vi "Main.vi"() -> ()   [LabVIEW 2020, in "DocTool.lvlib"]
uses:
  DocTool.lvlib
  TDefs/FP Items Properties Addendum.ctl
  TDefs/FP Items Properties.ctl
  TDefs/FP Item Properties.ctl
  TDefs/CopyTag.ctl
  TDefs/Single File Properties.ctl
  TDefs/Context.ctl
  Events/Events.ctl
  Events/UserEvent.ctl
  TDefs/State.ctl
  TDefs/States.ctl
  StateMachine.lvlib
panel:
  out "Status":string
  in  "Tab":enum32{"File Properties", "FP Items Properties"}(tab)
  out "Curr File":u16(slide) min=1 max=5 step=1 scale=1.0..5.0
  in  "Write FP":bool
  out "Total Files":u16
  in  "Copy_Desc":T1
  in  "Copy_HelpPath":T1
  in  "Copy_HelpTag":T1
  in  "File Properties":T2
  in  "PREV":bool
  in  "NEXT":bool
  in  "Read Folder":bool
  in  "Folder Path":path
  in  "SAVE":bool
  in  "Generate Help Tag":bool
  in  "Write":bool
  in  "Read File":bool
  out "FP VI Pic":picture
  out "BD VI Pic":picture
  in  "Connector Pane Terminals Only":bool
  in  "Tab Inputs":enum32{"Input", "More..."}(tab)
  in  "Inputs":T3
  in  "Input Addendum":T5
  in  "Tab Outputs":enum32{"Output", "More..."}(tab)
  in  "Outputs":T3
  in  "Output Addendum":T5
  in  "Mode":enum16{"All Items", "Selected Items"}(ring)
  in  "All":T1
  in  "Copy Descs to Tips":bool
  in  "Ignore Error Clusters":bool
  in  "Stop":bool
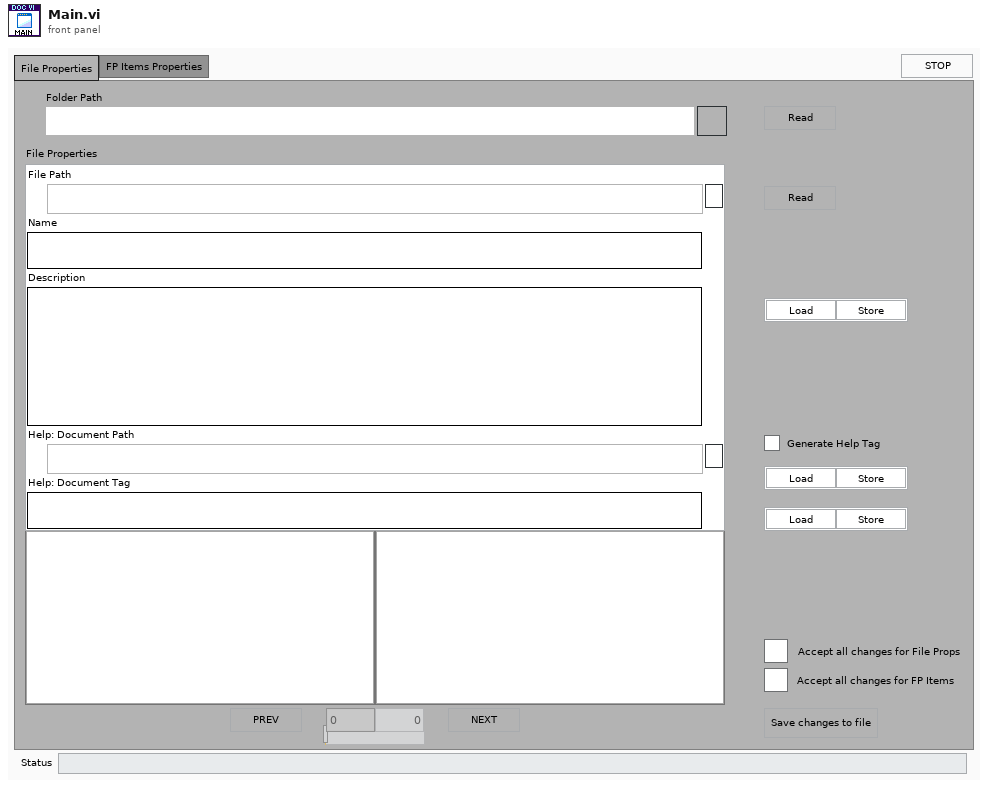
[diagram p1: front panel]
types:
  T1 = typedef "DocTool.lvlib/CopyTag.ctl" = cluster{"Load":bool, "Store":bool}
  T2 = typedef "DocTool.lvlib/Single File Properties.ctl" = cluster{"File Path":path, "Name":string, "Description":string, "Help: Document Path":path, "Help: Document Tag":string}
  T3 = typedef "DocTool.lvlib/FP Items Properties.ctl" = T4[]
  T4 = typedef "DocTool.lvlib/FP Item Properties.ctl" = cluster{"Sel":bool, "Idx":i32, "Name":string, "Description":string, "Tip":string, "Load Store":T1}
  T5 = typedef "DocTool.lvlib/FP Items Properties Addendum.ctl" = cluster{"Class Name":string[], "Class ID":dbl[]}
  T6 = typedef "DocTool.lvlib/Context.ctl" = cluster{"Events":T7, "States":cluster{"Current State":T9, "Next States":T10}, "General":cluster{"This VI":refnum<vi>, "Last Error":errorcluster}, "File":cluster{"Ref":refnum<vi>, "Props":T2, "Inputs":T3, "Outputs":T3, "Props Stored":T2, "Write":bool, "Write FP":bool, "Ignore Error Clusters":bool, "Copy Descs to Tips":bool, "CPTerminals Only":bool, "Generate Help Tag":bool}, "CtrlRefs":cluster{"File":cluster{"Properties":refnum<vi>, "Folder Path":refnum<vi>, "Read Folder":refnum<vi>, "Read File":refnum<vi>, "Path":refnum<vi>, "Help: Gen Tags":refnum<vi>, "Help: Doc Tag":refnum<vi>, "Help: Path":refnum<vi>}, "FP":cluster{"Inputs":refnum<vi>, "Outputs":refnum<vi>, "CP Terminals Only":refnum<vi>, "Ignore Error Clusters":refnum<vi>}, "Status":refnum<vi>, "Navigate":cluster{"Curr File":refnum<vi>, "NEXT":refnum<vi>, "PREV":refnum<vi>, "Total Files":refnum<vi>}}, "Folder":cluster{"Path":path, "File Paths":path[], "FilePath Index":i32}}
  T7 = typedef "StateMachine.lvlib/Events.ctl" = cluster{"Refnum":refnum<event-registration>, "Timeout":i32, "UserEvent":T8, "UserEvent Ref":refnum<user-event>}
  T8 = typedef "StateMachine.lvlib/UserEvent.ctl" = cluster{"ID":variant, "Data":variant}
  T9 = typedef "StateMachine.lvlib/State.ctl" = cluster{"ID":variant, "Data":variant}
  T10 = typedef "StateMachine.lvlib/States.ctl" = T9[]
  T11 = enum8{"Enabled", "Disabled", "Disabled and Grayed Out"}
  T12 = typedef "imagedata.ctl" = cluster{"image type":i32, "image depth":i32, "image":u8[], "mask":u8[], "colors":u32[], "Rectangle":cluster{"left":i16, "top":i16, "right":i16, "bottom":i16}}
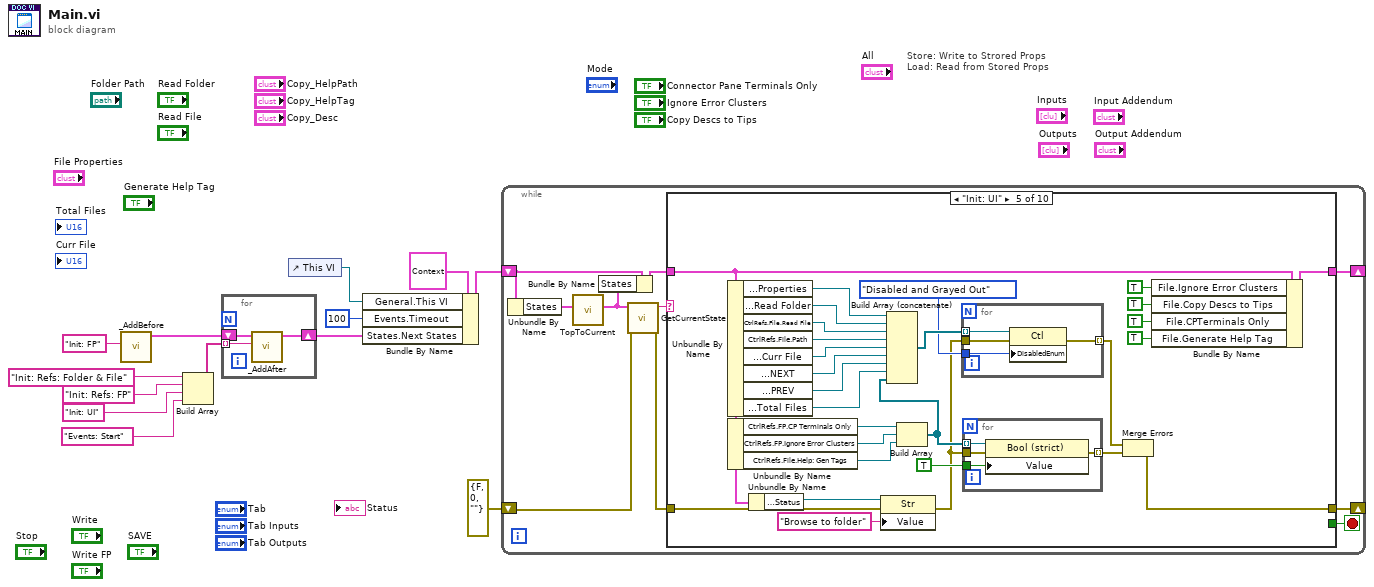
[diagram p0: block diagram]
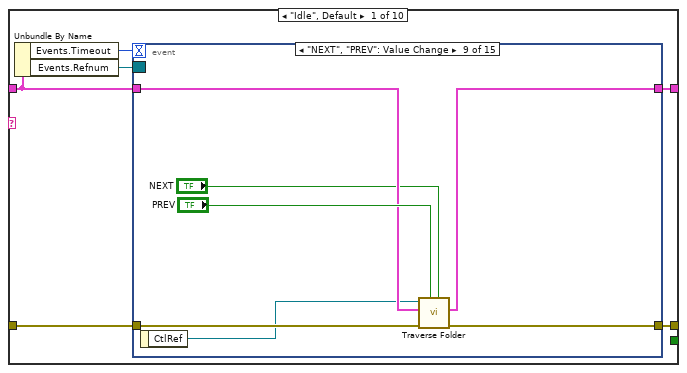
[diagram p2: hidden frame]
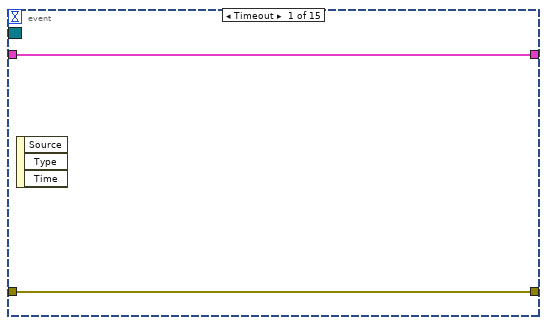
[diagram p3: hidden frame]
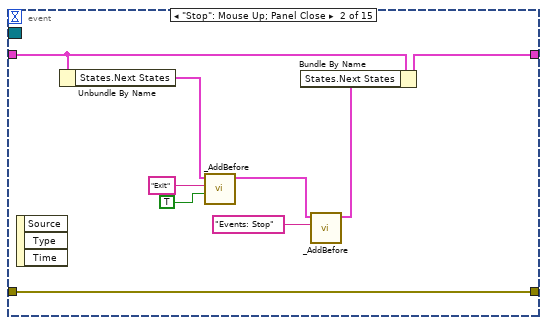
[diagram p4: hidden frame]
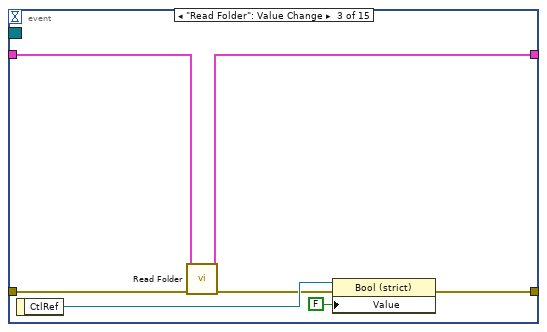
[diagram p5: hidden frame]
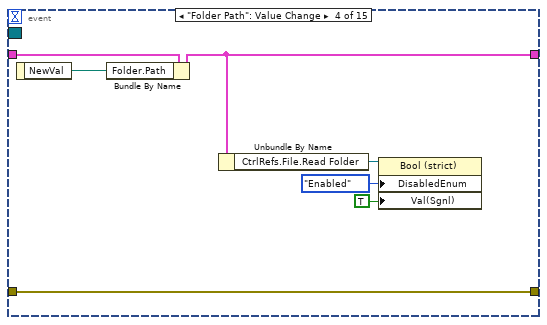
[diagram p6: hidden frame]
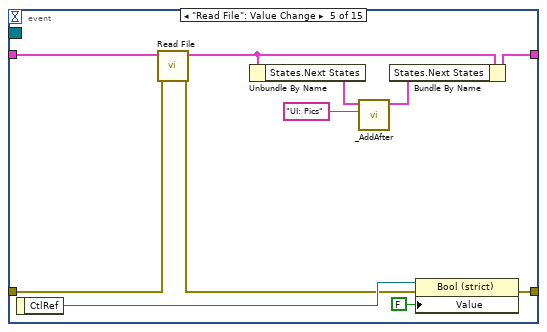
[diagram p7: hidden frame]
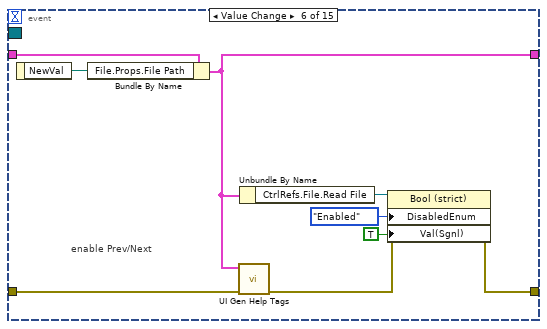
[diagram p8: hidden frame]
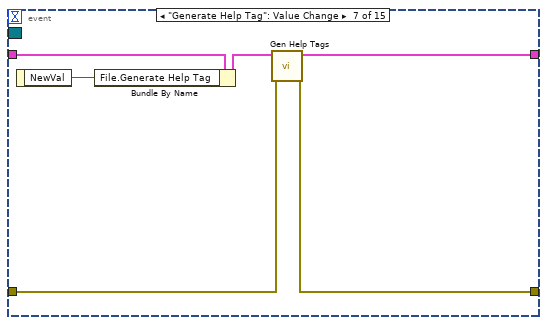
[diagram p9: hidden frame]
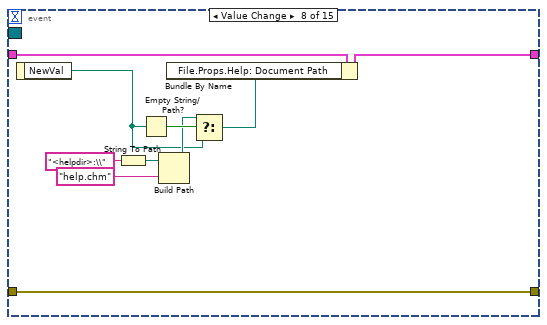
[diagram p10: hidden frame]
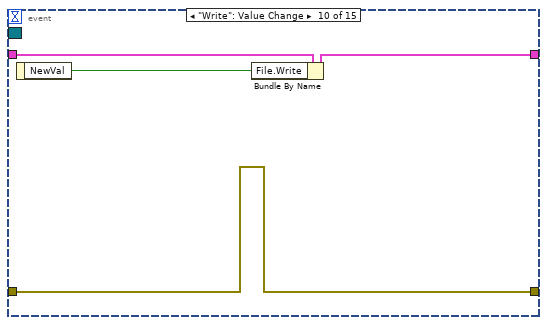
[diagram p11: hidden frame]
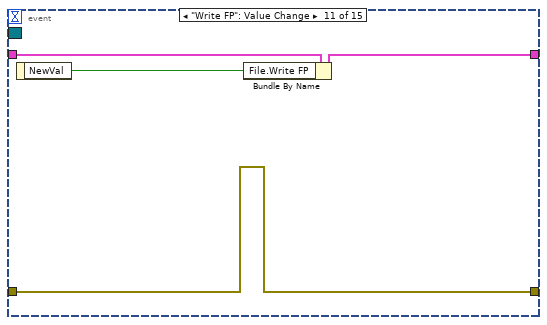
[diagram p12: hidden frame]
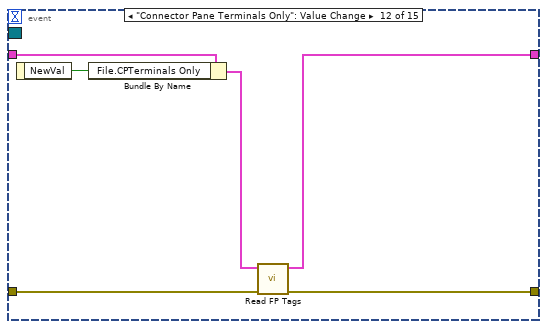
[diagram p13: hidden frame]
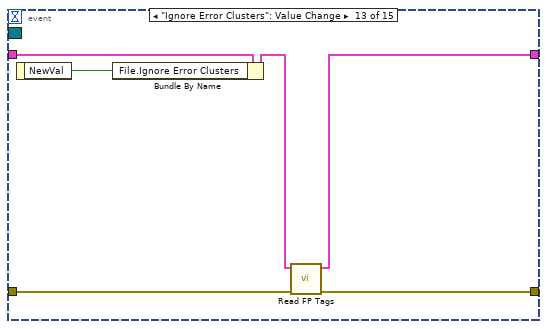
[diagram p14: hidden frame]
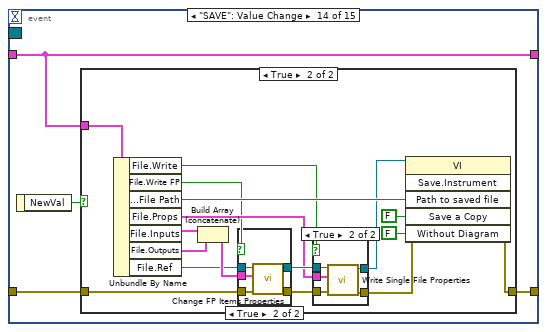
[diagram p15: hidden frame]
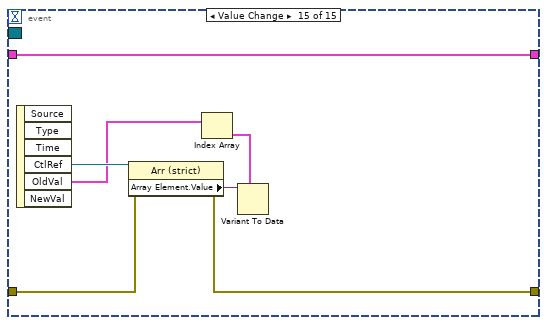
[diagram p19: hidden frame]
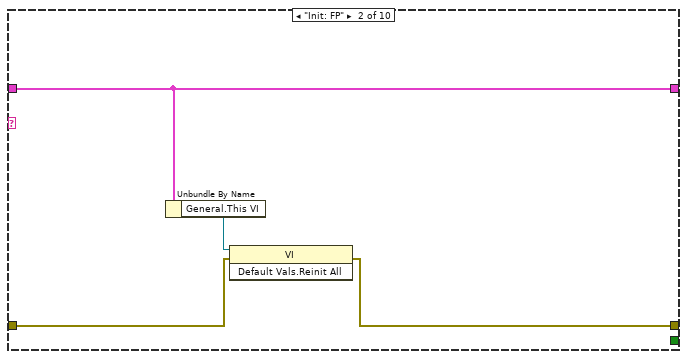
[diagram p20: hidden frame]
diagram:
  # "Store: Write to Strored Props\nLoad: Read from Stored Props"
  n1 = call "_AddBefore.vi"("ID"="Init: FP") -> ("Next States out"=w6:T10)  [unwired: 10 in]
  n2 = Build Array("Init: Refs: Folder & File", "Init: Refs: FP", "Init: UI", "Events: Start") -> (w1:string[])
  n3 = for {
    tunnel: w1 -> [w16] mode=indexing
    shift-right: [w15] -> w7
    shift-left: w6 -> [w14]
    n4 = call "_AddAfter.vi"("ID"=w16, "Next States in"=w14) -> ("Next States out"=w15:T10)  [unwired: 9 in]
  }
  n5 = control-ref of="This VI"() -> (w13:refnum<vi>)
  n6 = Bundle By Name(cluster=T6 {"Events"={"Refnum"=refnum, "Timeout"=0, "UserEvent"={"ID"=variant, "Data"=variant}, "UserEvent Ref"=refnum}, "States"={"Current State"={"ID"=variant, "Data"=variant}, "Next States"=[]}, "General"={"This VI"=refnum, "Last Error"={"status"=FALSE, "code"=0, "source"=""}}, "File"={"Ref"=refnum, "Props"={"File Path"=path "", "Name"="", "Description"="", "Help: Document Path"=path "", "Help: Document Tag"=""}, "Inputs"=[], "Outputs"=[], "Props Stored"={"File Path"=path "", "Name"="", "Description"="", "Help: Document Path"=path "", "Help: Document Tag"=""}, "Write"=FALSE, "Write FP"=FALSE, "Ignore Error Clusters"=FALSE, "Copy Descs to Tips"=FALSE, "CPTerminals Only"=FALSE, "Generate Help Tag"=FALSE}, "CtrlRefs"={"File"={"Properties"=refnum, "Folder Path"=refnum, "Read Folder"=refnum, "Read File"=refnum, "Path"=refnum, "Help: Gen Tags"=refnum, "Help: Doc Tag"=refnum, "Help: Path"=refnum}, "FP"={"Inputs"=refnum, "Outputs"=refnum, "CP Terminals Only"=refnum, "Ignore Error Clusters"=refnum}, "Status"=refnum, "Navigate"={"Curr File"=refnum, "NEXT"=refnum, "PREV"=refnum, "Total Files"=refnum}}, "Folder"={"Path"=path "", "File Paths"=[], "FilePath Index"=0}}, "General.This VI"=w13, "Events.Timeout"=100, "States.Next States"=w7) -> (w11:T6)
  n7 = while {
    shift-right: [w26] -> _
    shift-left: w11 -> [w22]
    shift-right: [w25] -> _
    shift-left: errorcluster {"status"=FALSE, "code"=0, "source"=""} ("error out") -> [w19]
    stop <- w24 stop-if-true
    n8 = Unbundle By Name(w22) -> ("States"=w17:cluster{"Current State":T9, "Next States":T10})
    n9 = call "TopToCurrent.vi"("States"=w17) -> ("States"=w18:cluster{"Current State":T9, "Next States":T10})  [unwired: 10 in]
    n10 = Bundle By Name(cluster=w22, "States"=w18) -> (w21:T6)
    n11 = call "GetCurrentState.vi"("error in (no error)"=w19, "States"=w18) -> ("error out"=w20:errorcluster, "Current State"=w23:string)  [unwired: 8 in]
    n12 = case shown="\"Init: UI\"" w23 {
      tunnel: w21 -> [w28 w164 w182 w190 w201 w237 w240 w248 w252 w260]
      tunnel: [w27 w164 w180 w189 w214 w237 w240 w248 w252 w261] -> w26
      tunnel: w20 -> [w29 w166 w181 w186 w198 w238 w242 w244 w249 w257]
      tunnel: [w30 w165 w181 w186 w207 w227 errorcluster {"status"=FALSE, "code"=0, "source"=""} ("error out") w245 w253 w262] -> w25
      tunnel: [_ _ _ _ _ _ _ w243 _ _] -> w24
      frame "Idle", Default {
        n13 = Unbundle By Name(w28) -> ("Events.Timeout"=w31:i32, "Events.Refnum"=w32:refnum<event-registration>)
        n14 = event shown="[8] \"NEXT\", \"PREV\": Value Change" {
          selector: w32 -> [_ _ _ _ _ _ _ _ _ _ _ _ _ _ _]
          dyn-events: _ -> [_ _ _ _ _ _ _ _ _ _ _ _ _ _ _]
          timeout: w31 -> [_ _ _ _ _ _ _ _ _ _ _ _ _ _ _]
          tunnel: [w34 w43 w44 w57 w64 w69 w80 w93 w96 w103 w107 w109 w118 w123 w161] -> w30
          tunnel: w29 -> [w34 w43 w50 w57 w68 w71 w81 w93 w100 w103 w107 w110 w117 w124 w162]
          tunnel: w28 -> [w33 w39 w48 w56 w67 w77 w83 w92 w98 w104 w108 w114 w120 w122 w160]
          tunnel: [w33 w40 w49 w54 w59 w72 w82 w91 w95 w102 w106 w111 w115 w122 w160] -> w27
          event Timeout {
            n15 = event-data() -> ()  [unwired: 1 in, 3 out]
          }
          event "Stop": Mouse Up; Panel Close {
            n16 = event-data() -> ()  [unwired: 1 in, 3 out]
            n17 = Unbundle By Name(w39) -> ("States.Next States"=w36:T10)
            n18 = call "_AddBefore.vi"("Data"=TRUE, "ID"="Exit", "Next States in"=w36) -> ("Next States out"=w37:T10)  [unwired: 8 in]
            n19 = call "_AddBefore.vi"("ID"="Events: Stop", "Next States in"=w37) -> ("Next States out"=w35:T10)  [unwired: 9 in]
            n20 = Bundle By Name(cluster=w39, "States.Next States"=w35) -> (w40:T6)
          }
          event "Read Folder": Value Change {
            n21 = event-data() -> ("CtlRef"=w46:refnum<vi>)  [unwired: 1 in]
            n22 = call "Read Folder.vi"("error in (no error)"=w50, "Context in"=w48) -> ("error out"=w45:errorcluster, "Context out"=w49:T6)  [unwired: 8 in]
            n23 = property class="Bool (strict)"(reference=w46, error in=w45, "Value"=FALSE) -> (error out=w44:errorcluster)  [unwired: 1 out]
          }
          event "Folder Path": Value Change {
            n24 = event-data() -> ("NewVal"=w55:path)  [unwired: 1 in]
            n25 = Bundle By Name(cluster=w56, "Folder.Path"=w55) -> (w54:T6)
            n26 = Unbundle By Name(w54) -> ("CtrlRefs.File.Read Folder"=w53:refnum<vi>)
            n27 = property class="Bool (strict)"(reference=w53, "DisabledEnum"=T11."Enabled" ("Disabled"), "Val(Sgnl)"=TRUE ("Value (Signaling)")) -> ()  [unwired: 1 in, 2 out]
          }
          event "Read File": Value Change {
            n28 = event-data() -> ("CtlRef"=w65:refnum<vi>)  [unwired: 1 in]
            n29 = call "Read File.vi"("error in (no error)"=w68, "Context in"=w67) -> ("error out"=w63:errorcluster, "Context out"=w60:T6)  [unwired: 8 in]
            n30 = Unbundle By Name(w60) -> ("States.Next States"=w62:T10)
            n31 = call "_AddAfter.vi"("ID"="UI: Pics", "Next States in"=w62) -> ("Next States out"=w61:T10)  [unwired: 9 in]
            n32 = Bundle By Name(cluster=w60, "States.Next States"=w61) -> (w59:T6)
            n33 = property class="Bool (strict)"(reference=w65, error in=w63, "Value"=FALSE) -> (error out=w64:errorcluster)  [unwired: 1 out]
          }
          event Value Change {
            # "enable Prev/Next"
            n34 = event-data() -> ("NewVal"=w76:path)  [unwired: 1 in]
            n35 = Bundle By Name(cluster=w77, "File.Props.File Path"=w76) -> (w72:T6)
            n36 = call "UI Gen Help Tags.vi"("error in (no error)"=w71, "Context"=w72) -> ("error out"=w70:errorcluster)  [unwired: 9 in]
            n37 = Unbundle By Name(w72) -> ("CtrlRefs.File.Read File"=w75:refnum<vi>)
            n38 = property class="Bool (strict)"(reference=w75, error in=w70, "DisabledEnum"=T11."Enabled" ("Disabled"), "Val(Sgnl)"=TRUE ("Value (Signaling)")) -> (error out=w69:errorcluster)  [unwired: 1 out]
          }
          event "Generate Help Tag": Value Change {
            n39 = event-data() -> ("NewVal"=w78:bool)  [unwired: 1 in]
            n40 = Bundle By Name(cluster=w83, "File.Generate Help Tag"=w78) -> (w79:T6)
            n41 = call "Gen Help Tags.vi"("error in (no error)"=w81, "Context in"=w79) -> ("error out"=w80:errorcluster, "Context out"=w82:T6)  [unwired: 8 in]
          }
          event Value Change {
            n42 = event-data() -> ("NewVal"=w85:path)  [unwired: 1 in]
            n43 = String To Path(string="<helpdir>:\\") -> (path=w88:path)
            n44 = Empty String/Path?(string/path=w85) -> (empty?=w87:bool)
            n45 = Build Path(base path=w88, name or relative path="help.chm") -> (appended path=w86:path)
            n46 = Select(t=w86, s=w87, f=w85) -> (s? t:f=w84:path)
            n47 = Bundle By Name(cluster=w92, "File.Props.Help: Document Path"=w84) -> (w91:T6)
          }
          event "NEXT", "PREV": Value Change {
            n48 = event-data() -> ("CtlRef"=w97:refnum<vi>)  [unwired: 1 in]
            n49 = call "Traverse Folder.vi"("NEXT"="NEXT", "PREV"="PREV", "error in (no error)"=w100, "Context"=w98, "Boolean in"=w97) -> ("error out"=w96:errorcluster, "Context out"=w95:T6)  [unwired: 5 in]
          }
          event "Write": Value Change {
            n50 = event-data() -> ("NewVal"=w101:bool)  [unwired: 1 in]
            n51 = Bundle By Name(cluster=w104, "File.Write"=w101) -> (w102:T6)
          }
          event "Write FP": Value Change {
            n52 = event-data() -> ("NewVal"=w105:bool)  [unwired: 1 in]
            n53 = Bundle By Name(cluster=w108, "File.Write FP"=w105) -> (w106:T6)
          }
          event "Connector Pane Terminals Only": Value Change {
            n54 = event-data() -> ("NewVal"=w113:bool)  [unwired: 1 in]
            n55 = Bundle By Name(cluster=w114, "File.CPTerminals Only"=w113) -> (w112:T6)
            n56 = call "Read FP Tags.vi"("error in (no error)"=w110, "Context in"=w112) -> ("error out"=w109:errorcluster, "Context out"=w111:T6)  [unwired: 8 in]
          }
          event "Ignore Error Clusters": Value Change {
            n57 = event-data() -> ("NewVal"=w119:bool)  [unwired: 1 in]
            n58 = Bundle By Name(cluster=w120, "File.Ignore Error Clusters"=w119) -> (w116:T6)
            n59 = call "Read FP Tags.vi"("error in (no error)"=w117, "Context in"=w116) -> ("error out"=w118:errorcluster, "Context out"=w115:T6)  [unwired: 8 in]
          }
          event "SAVE": Value Change {
            n60 = event-data() -> ("NewVal"=w121:bool)  [unwired: 1 in]
            n61 = case shown="True" w121 {
              tunnel: w124 -> [w125 w130]
              tunnel: [w125 w139] -> w123
              tunnel: w122 -> [_ w138]
              frame False {
              }
              frame True {
                n62 = Unbundle By Name(w138) -> ("File.Write"=w126:bool, "File.Write FP"=w127:bool, "File.Props.File Path"=w140:path, "File.Props"=w132:T2, "File.Inputs"=w137:T3, "File.Outputs"=w136:T3, "File.Ref"=w131:refnum<vi>)
                n63 = Build Array (concatenate)(w137, w136) -> (w135:T3)
                n64 = case shown="True" w127 {
                  tunnel: w135 -> [_ w156]
                  tunnel: [w151 w155] -> w134
                  tunnel: w131 -> [w151 w154]
                  tunnel: w130 -> [w150 w153]
                  tunnel: [w150 w152] -> w129
                  frame False {
                  }
                  frame True {
                    n65 = call "Change FP Items Properties.vi"("error in (no error)"=w153, "Input + Output"=w156, "VI in"=w154) -> ("error out"=w152:errorcluster, "VI out"=w155:refnum<vi>)  [unwired: 7 in]
                  }
                }
                n66 = case shown="True" w126 {
                  tunnel: w134 -> [w143 w149]
                  tunnel: [w143 w148] -> w133
                  tunnel: w132 -> [_ w147]
                  tunnel: w129 -> [w144 w146]
                  tunnel: [w144 w145] -> w128
                  frame False {
                  }
                  frame True {
                    n67 = call "Write Single File Properties.vi"("error in (no error)"=w146, "File Properties in"=w147, "VI"=w149) -> ("error out"=w145:errorcluster, "VI out"=w148:refnum<vi>)  [unwired: 7 in]
                  }
                }
                n68 = invoke class="VI" method="Save.Instrument"(reference=w133, error in=w128, "Path to saved file"=w140, "Save a Copy"=FALSE, "Without Diagram"=FALSE) -> (error out=w139:errorcluster)  [unwired: 1 in, 5 out]
              }
            }
          }
          event Value Change {
            n69 = event-data() -> ("CtlRef"=w163:refnum<vi>, "OldVal"=w158:T3)  [unwired: 1 in, 4 out]
            n70 = property class="Arr (strict)"(reference=w163, error in=w162) -> (error out=w161:errorcluster, "Array Element.Value"=w159:variant)  [unwired: 1 out]
            n71 = Index Array(array=w158) -> (element=w157:T4)  [unwired: 1 in]
            n72 = Variant To Data(type=w157, Variant=w159) -> ()  [unwired: 1 in, 2 out]
          }
        }
      }
      frame "Init: FP" {
        n73 = Unbundle By Name(w164) -> ("General.This VI"=w167:refnum<vi>)
        n74 = invoke class="VI" method="Default Vals.Reinit All"(reference=w167, error in=w166) -> (error out=w165:errorcluster)  [unwired: 1 in, 2 out]
      }
      frame "Init: Refs: Folder & File" {
        n75 = control-ref of="Read Folder"() -> (w177:refnum<vi>)
        n76 = control-ref of="Read File"() -> (w176:refnum<vi>)
        n77 = control-ref of="Generate Help Tag"() -> (w174:refnum<vi>)
        n78 = control-ref of="NEXT"() -> (w169:refnum<vi>)
        n79 = control-ref of="PREV"() -> (w168:refnum<vi>)
        n80 = control-ref of="File Properties"() -> (w179:refnum<vi>)
        n81 = control-ref of="Total Files"() -> (w170:refnum<vi>)
        n82 = control-ref of="Help: Document Tag"() -> (w173:refnum<vi>)
        n83 = control-ref of="Folder Path"() -> (w178:refnum<vi>)
        n84 = control-ref of="File Path"() -> (w175:refnum<vi>)
        n85 = control-ref of="Help: Document Path"() -> (w172:refnum<vi>)
        n86 = control-ref of="Curr File"() -> (w171:refnum<vi>)
        n87 = Bundle By Name(cluster=w182, "CtrlRefs.File.Properties"=w179, "CtrlRefs.File.Folder Path"=w178, "CtrlRefs.File.Read Folder"=w177, "CtrlRefs.File.Read File"=w176, "CtrlRefs.File.Path"=w175, "CtrlRefs.File.Help: Gen Tags"=w174, "CtrlRefs.File.Help: Doc Tag"=w173, "CtrlRefs.File.Help: Path"=w172, "CtrlRefs.Navigate.Curr File"=w171, "CtrlRefs.Navigate.Total Files"=w170, "CtrlRefs.Navigate.NEXT"=w169, "CtrlRefs.Navigate.PREV"=w168) -> (w180:T6)
      }
      frame "Init: Refs: FP" {
        n88 = control-ref of="Connector Pane Terminals Only"() -> (w185:refnum<vi>)
        n89 = control-ref of="Ignore Error Clusters"() -> (w184:refnum<vi>)
        n90 = control-ref of="Status"() -> (w183:refnum<vi>)
        n91 = control-ref of="Inputs"() -> (w188:refnum<vi>)
        n92 = control-ref of="Outputs"() -> (w187:refnum<vi>)
        n93 = Bundle By Name(cluster=w190, "CtrlRefs.FP.Inputs"=w188, "CtrlRefs.FP.Outputs"=w187, "CtrlRefs.FP.CP Terminals Only"=w185, "CtrlRefs.FP.Ignore Error Clusters"=w184, "CtrlRefs.Status"=w183) -> (w189:T6)
      }
      frame "Init: UI" {
        n94 = Unbundle By Name(w201) -> ("CtrlRefs.File.Properties"=w191:refnum<vi>, "CtrlRefs.File.Read Folder"=w218:refnum<vi>, "CtrlRefs.File.Read File"=w216:refnum<vi>, "CtrlRefs.File.Path"=w196:refnum<vi>, "CtrlRefs.Navigate.Curr File"=w195:refnum<vi>, "CtrlRefs.Navigate.NEXT"=w194:refnum<vi>, "CtrlRefs.Navigate.PREV"=w193:refnum<vi>, "CtrlRefs.Navigate.Total Files"=w192:refnum<vi>)
        n95 = Unbundle By Name(w201) -> ("CtrlRefs.FP.CP Terminals Only"=w211:refnum<vi>, "CtrlRefs.FP.Ignore Error Clusters"=w210:refnum<vi>, "CtrlRefs.File.Help: Gen Tags"=w203:refnum<vi>)
        n96 = Unbundle By Name(w201) -> ("CtrlRefs.Status"=w200:refnum<vi>)
        n97 = property class="Str"(reference=w200, error in=w198, "Value"="Browse to folder") -> (error out=w199:errorcluster)  [unwired: 1 out]
        n98 = Build Array(w211, w210, w203) -> (w202:refnum<vi>[])
        n99 = Build Array (concatenate)(w191, w218, w216, w196, w195, w194, w193, w192, w202) -> (w217:refnum<vi>[])
        n100 = for {
          tunnel: w217 -> [w226] mode=indexing
          tunnel: w199 -> [w225]
          tunnel: [w224] -> w206 mode=indexing
          tunnel: T11."Disabled and Grayed Out" ("Disabled") -> [w223]
          n101 = property class="Ctl"(reference=w226, error in=w225, "DisabledEnum"=w223) -> (error out=w224:errorcluster)  [unwired: 1 out]
        }
        n102 = for {
          tunnel: w202 -> [w222] mode=indexing
          tunnel: [w221] -> w208 mode=indexing
          tunnel: TRUE ("File.Copy Descs to Tips") -> [w220]
          tunnel: w199 -> [w219]
          n103 = property class="Bool (strict)"(reference=w222, error in=w219, "Value"=w220) -> (error out=w221:errorcluster)  [unwired: 1 out]
        }
        n104 = Merge Errors(w206, w208) -> (w207:errorcluster)
        n105 = Bundle By Name(cluster=w201, "File.Ignore Error Clusters"=TRUE, "File.Copy Descs to Tips"=TRUE, "File.CPTerminals Only"=TRUE, "File.Generate Help Tag"=TRUE) -> (w214:T6)
      }
      frame "UI: Pics" {
        n106 = Unbundle By Name(w237) -> ("File.Ref"=w236:refnum<vi>)
        n107 = invoke class="VI" method="Get Conpane Image"(reference=w236, error in=w238) -> (reference out=w229:refnum<vi>, error out=w228:errorcluster, "Get Conpane Image"=w239:T12)  [unwired: 1 in]
        n108 = invoke class="VI" method="BD.Get Image Scaled"(reference=w229, error in=w228, "img depth"=8 ("Image Depth"), "max width"=350 ("Maximum Width"), "max height"=175 ("Maximum Height")) -> (error out=w227:errorcluster, "img data"=w230:T12)  [unwired: 2 in, 5 out]
        n109 = call <vilib>:"Draw Flattened Pixmap.vi"("image data"=w230) -> ("new picture"=→"BD VI Pic":picture)  [unwired: 8 in]
        n110 = call <vilib>:"Draw Flattened Pixmap.vi"("image data"=w239) -> ("new picture"=→"FP VI Pic":picture)  [unwired: 8 in]
      }
      frame "Error" {
        n111 = call <vilib>:"Simple Error Handler.vi"("error in (no error)"=w242) -> ()  [unwired: 4 in, 5 out]
      }
      frame "Exit" {
        n112 = Unbundle By Name(w248) -> ("States.Current State.Data"=w247:variant)
        n113 = Variant To Data(error in=w244, type=FALSE, Variant=w247) -> (data=w243:bool, error out=w245:errorcluster)
      }
      frame "Events: Stop" {
        n114 = Unbundle By Name(w252) -> ("Events.Refnum"=w254:refnum<event-registration>, "Events.UserEvent Ref"=w251:refnum<user-event>)
        n115 = Destroy User Event(user event=w251, error in=w249) -> (error out=w250:errorcluster)
        n116 = Unregister For Events(event registration refnum=w254, error in=w250) -> (error out=w253:errorcluster)
      }
      frame "Events: Start" {
        n117 = Unbundle By Name(w260) -> ("Events.UserEvent"=w259:T8)
        n118 = Create User Event(user event datatype=w259, error in=w257) -> (user event=w255:refnum<user-event>, error out=w256:errorcluster)
        n119 = register-events(error in=w256, w255) -> (reference out=w258:refnum<event-registration>, error out=w262:errorcluster)  [unwired: 1 in]
        n120 = Bundle By Name(cluster=w260, "Events.UserEvent Ref"=w255, "Events.Refnum"=w258) -> (w261:T6)
      }
    }
  }
